vi "- VI Tree - Command-Line Zip.vi"() -> ()   [LabVIEW 2019]
uses:
  Command-Line Zip.lvlib
panel:
  in  "Boolean":bool
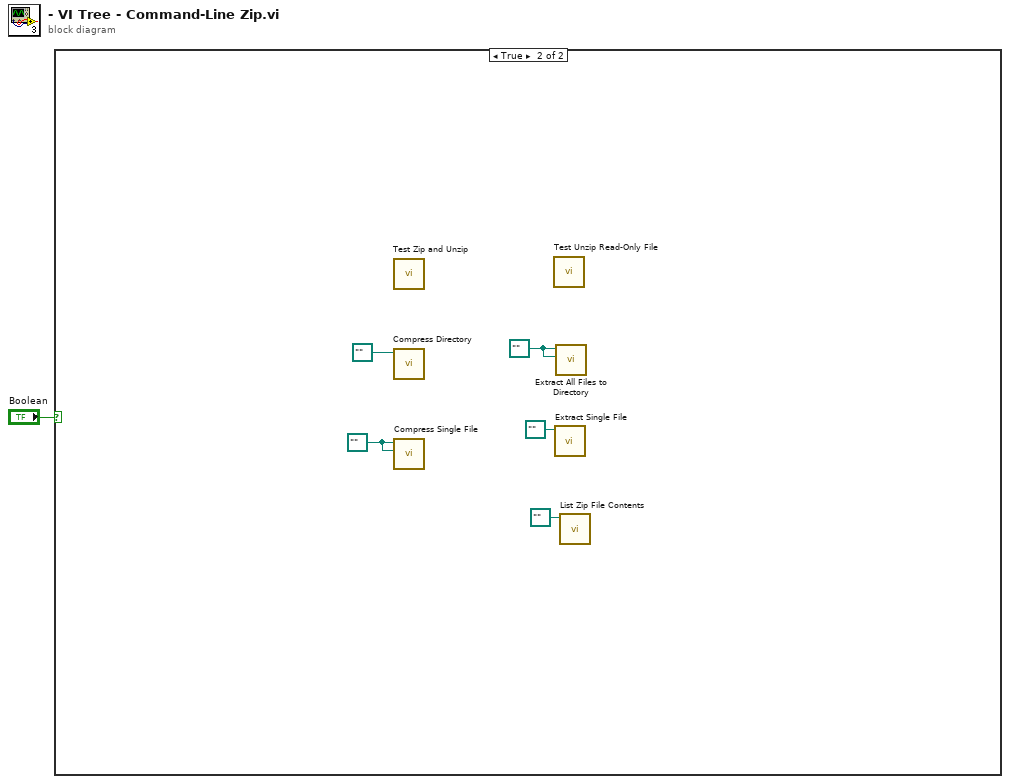
[diagram p0: block diagram]
diagram:
  n1 = case shown="True" "Boolean" {
    frame False {
    }
    frame True {
      w4 = path "" ("Zip File Path")
      w5 = path "" ("Zip File Path")
      n2 = call "Test Zip and Unzip.vi"() -> ()  [unwired: 12 in]
      n3 = call "Compress Directory.vi"("root directory (file dialog)"=path "") -> ()  [unwired: 8 in, 3 out]
      n4 = call "Compress Single File.vi"("Source File Path"=w5, "Zip File Path"=w5) -> ()  [unwired: 7 in, 3 out]
      n5 = call "Test Unzip Read-Only File.vi"() -> ()  [unwired: 12 in]
      n6 = call "Extract Single File.vi"("Zip File Path"=path "") -> ()  [unwired: 7 in, 4 out]
      n7 = call "Extract All Files to Directory.vi"("Extract to Dir"=w4, "Zip File Path"=w4) -> ()  [unwired: 9 in, 1 out]
      n8 = call "List Zip File Contents.vi"("Zip File Path"=path "" ("Package File Path")) -> ()  [unwired: 6 in, 5 out]
    }
  }
